vi "Vertical speed (SubVI).vi"(8 "error in (no error)":errorcluster, 11 "Array of Joint Positions in":dbl[][](array[numeric])=[[-0.12146424502134323, 0.001454623183235526, 1.9073543548583984], [-0.11488837748765945, 0.05537768453359604, 1.9802660942077637], [-0.11157815903425217, 0.43785253167152405, 2.0466103553771973], [-0.1483002007007599, 0.6516268253326416, 2.0609679222106934], [-0.30285415053367615, 0.2956160008907318, 2.029113531112671], [-0.38003623485565186, 0.031045880168676376, 1.9445093870162964], [-0.35092946887016296, -0.1451244205236435, 1.7685273885726929], [-0.3320053219795227, -0.2223913073539734, 1.670140027999878], [0.04304381087422371, 0.29154613614082336, 1.9958680868148804], [0.13985766470432281, 0.025840533897280693, 1.922817349433899], [0.12575246393680573, -0.14097267389297485, 1.7425767183303833], [0.10289721190929413, -0.2135094851255417, 1.649812936782837], [-0.1967616081237793, -0.07389465719461441, 1.8869941234588623], [-0.2406357079744339, -0.5076637864112854, 1.838017225265503], [-0.23708361387252808, -0.8213208913803101, 1.8209781646728516], [-0.24613811075687408, -0.8672351241111755, 1.7265561819076538], [-0.04989041015505791, -0.0703207477927208, 1.876594066619873], [-0.015257264487445354, -0.5077733993530273, 1.839611291885376], [-0.002423219382762909, -0.818880021572113, 1.8193140029907227], [-0.007616172078996897, -0.8644676804542542, 1.7244435548782349]]) -> (0 "error out":errorcluster, 2 "hands are at same alt":bool, 3 "Vertical Speed":dbl)   [LabVIEW 2014]
uses:
  <vilib>/Analysis/NI_AALPro.lvlib
panel:
  in  "Method":bool
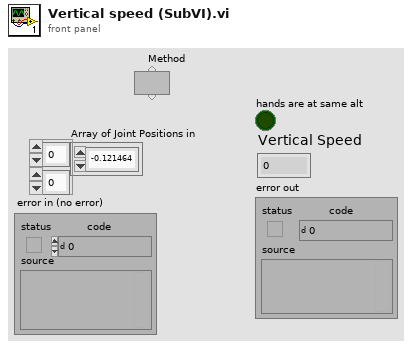
[diagram p1: front panel]
types:
  T1 = enum16{"hip centre", "spine", "shoulder centre", "head", "shoulder left", "elbow left", "wrist left", "hand left", "shoulder right", "elbow right", "wrist right", "hand right", "hip left", "knee left", "ankle left", "foot left", "hip right", "knee right", "ankle right", "foot right"}
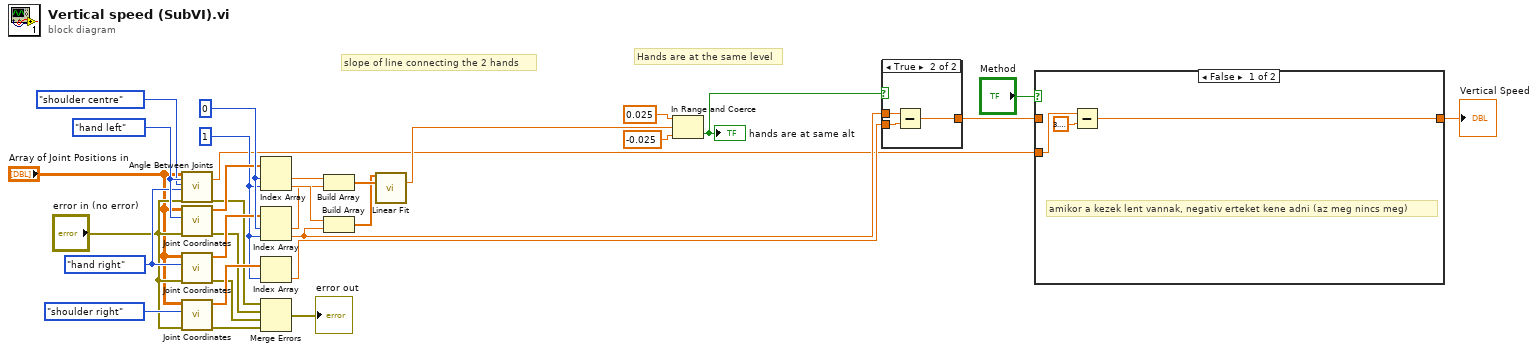
[diagram p0: block diagram]
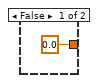
[diagram p3: hidden frame]
diagram:
  w16 = 1 ("index")
  w31 = 0 ("index")
  w8 = T1."hand right" ("Joint 2")
  w10 = T1."hand left" ("Joint 1")
  # "Hands are at the same level"
  # "slope of line connecting the 2 hands"
  n1 = call <vilib>:"Angle Between Joints.vi"("Array of Joint Positions"="Array of Joint Positions in", "Joint 1"=w10, "Joint 2"=T1."shoulder centre", "Joint 3"=w8, "error in (no error)"="error in (no error)") -> ("Angle Between Joints (rads)"=w1:dbl, "error out"=w6:errorcluster)  [unwired: 9 in, 4 out]
  n2 = call <vilib>:"Joint Coordinates.vi"("error in (no error)"="error in (no error)", "Joint 1"=w10, "Array of Joint Positions"="Array of Joint Positions in") -> ("error out"=w11:errorcluster, "Joint Coordinates"=w28:dbl[])  [unwired: 7 in]
  n3 = call <vilib>:"Joint Coordinates.vi"("error in (no error)"="error in (no error)", "Joint 1"=w8, "Array of Joint Positions"="Array of Joint Positions in") -> ("error out"=w12:errorcluster, "Joint Coordinates"=w29:dbl[])  [unwired: 7 in]
  n4 = call <vilib>:"Joint Coordinates.vi"("error in (no error)"="error in (no error)", "Joint 1"=T1."shoulder right" ("Joint 2"), "Array of Joint Positions"="Array of Joint Positions in") -> ("error out"=w13:errorcluster, "Joint Coordinates"=w30:dbl[])  [unwired: 7 in]
  n5 = Index Array(array=w28, index #1=w31, index #2=w16) -> (element #1=w26:dbl, element #2=w25:dbl)
  n6 = Index Array(array=w29, index #1=w31, index #2=w16) -> (element #1=w19:dbl, element #2=w15:dbl)
  n7 = Index Array(array=w30, index=w16) -> (element=w18:dbl)
  n8 = Merge Errors(w6, w11, w12, w13) -> (→"error out":errorcluster)
  n9 = Build Array(w26, w19) -> (w24:dbl[])
  n10 = Build Array(w25, w15) -> (w23:dbl[])
  n11 = call <vilib>:"Linear Fit.vi"("Y"=w23, "X"=w24) -> ("slope"=w22:dbl)  [unwired: 9 in, 4 out]
  n12 = In Range and Coerce(upper limit=0.025, x=w22, lower limit=-0.025) -> (In Range?=w17:bool)  [unwired: 1 out]
  "hands are at same alt" <- w17
  n13 = case shown="True" w17 {
    tunnel: w15 -> [_ w35]
    tunnel: w18 -> [_ w34]
    tunnel: [0.0 w33] -> w3
    frame False {
    }
    frame True {
      n14 = Subtract(x=w35, y=w34) -> (x-y=w33:dbl)
    }
  }
  n15 = case shown="False" "Method" {
    tunnel: [w36 w39] -> w2
    tunnel: w3 -> [_ w39]
    tunnel: w1 -> [w38 _]
    frame False {
      # "amikor a kezek lent vannak, negativ erteket kene adni (az meg nincs meg)"
      n16 = Subtract(x=w38, y=3.141592653589793) -> (x-y=w36:dbl)
    }
    frame True {
    }
  }
  "Vertical Speed" <- w2
